vi "Create Numeric Channel.vi"(7 "Input?":bool, 8 "error in (no error)":errorcluster, 10 "Channel Number":i32) -> (0 "error out":errorcluster, 2 "Numeric Channel":T1, 3 "Channel out":refnum<class "Channel.lvclass">)   [LabVIEW 2026, in "Modbus.lvlib" / "Modbus.lvclass"]
uses:
  Modbus.lvclass
  <vilib>/FlexLogger/SDK/PluginSDK.lvlibp/PEFClasses/SDK/Channel/Channel.lvclass
  Types/Numeric Data.ctl
  Types/Modbus Table.ctl
  Types/Numeric Size.ctl
  Types/Numeric Data Type.ctl
  Types/Numeric Location.ctl
  1585c66d-b047-40a8-b383-e25739784f18.vi
  2dd19376-ff6e-472a-aab6-17888e896a0b.vi
  e0cdf0dc-ec87-4ce3-9d59-fa7e6132dbb7.vi
  2dd19376-ff6e-472a-aab6-17888e896a0b.vi/407e0540-03f6-4363-afc5-a4b1f046ef19.vi
  2dd19376-ff6e-472a-aab6-17888e896a0b.vi/520d475a-7b95-4b20-931b-ccc2be82a762.vi
  <vilib>/FlexLogger/SDK/PluginSDK.lvlibp/PEFClasses/SDK/Setpoint Consumer Channel/Setpoint Consumer Channel.lvclass
  <vilib>/FlexLogger/SDK/PluginSDK.lvlibp/PEFClasses/SDK/Producer Channel/Producer Channel.lvclass
  Globals/Modbus Strings.vi
  <vilib>/FlexLogger/SDK/PluginSDK.lvlibp/PEFClasses/SDK/Setpoint Consumer Channel/Create Setpoint Consumer Channel_v2.vi
  <vilib>/FlexLogger/SDK/PluginSDK.lvlibp/PEFClasses/SDK/Producer Channel/Create Producer Channel_v2.vi
  <vilib>/FlexLogger/SDK/PluginSDK.lvlibp/PEFClasses/SDK/Channel/ParameterAccess/Write Enum.vi
  <vilib>/FlexLogger/SDK/PluginSDK.lvlibp/PEFClasses/SDK/Channel/ParameterAccess/Write I32.vi
  <vilib>/FlexLogger/SDK/PluginSDK.lvlibp
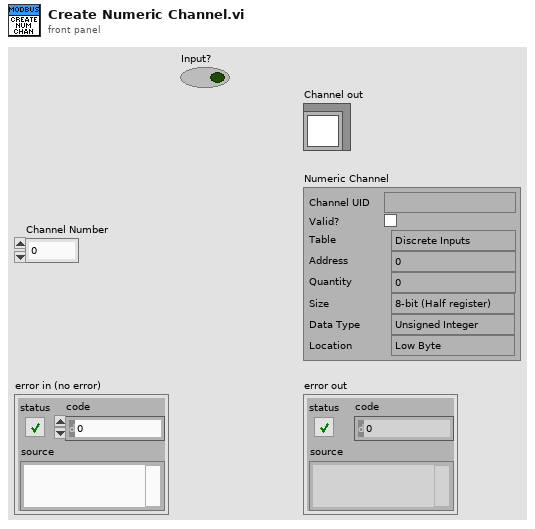
[diagram p1: front panel]
types:
  T1 = typedef "Modbus.lvlib/Modbus.lvclass/Numeric Data.ctl" = cluster{"Channel UID":string, "Valid?":bool, "Table":T2, "Address":i32, "Quantity":u16, "Size":T3, "Data Type":T4, "Location":T5}
  T2 = typedef "Modbus.lvlib/Modbus.lvclass/Modbus Table.ctl" = enum16{"Discrete Inputs", "Coils", "Input Registers", "Holding Registers"}
  T3 = typedef "Modbus.lvlib/Modbus.lvclass/Numeric Size.ctl" = enum16{"8-bit (Half register)", "16-bit (One register)", "32-bit (Two registers)", "64-bit (Four registers)"}
  T4 = typedef "Modbus.lvlib/Modbus.lvclass/Numeric Data Type.ctl" = enum16{"Unsigned Integer", "Signed Integer", "Floating Point"}
  T5 = typedef "Modbus.lvlib/Modbus.lvclass/Numeric Location.ctl" = enum16{"Low Byte", "High Byte"}
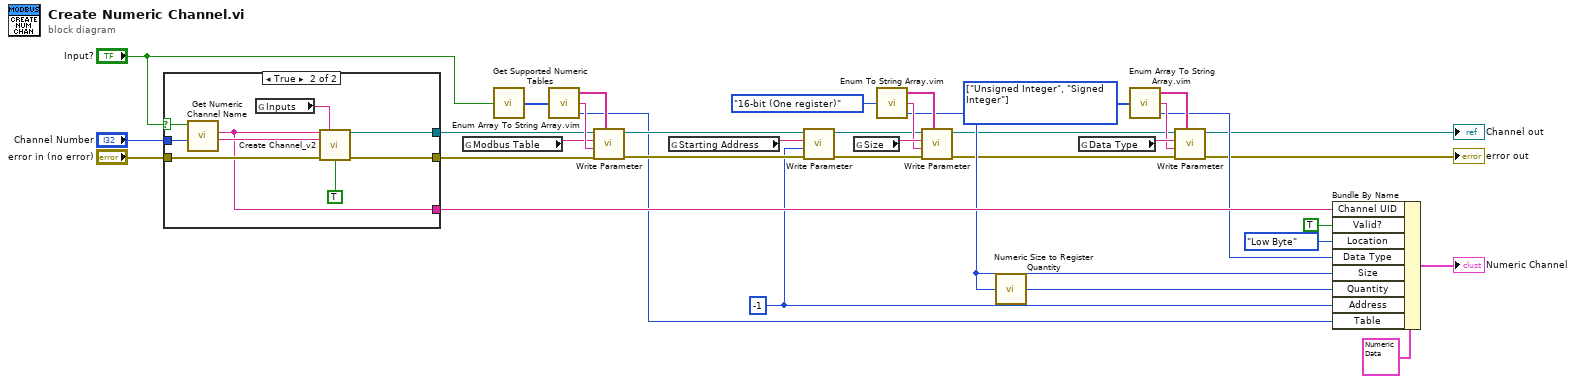
[diagram p0: block diagram]
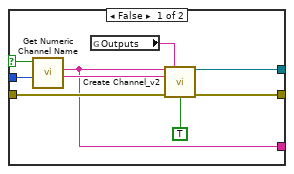
[diagram p2: hidden frame]
diagram:
  w4 = T4[] [enum."Unsigned Integer", enum."Signed Integer"] items=["Unsigned Integer", "Signed Integer", "Floating Point"]
  w20 = -1 ("Value")
  n1 = case shown="True" "Input?" {
    selector: "Input?" -> [w40 w49]
    tunnel: "error in (no error)" -> [w42 w51]
    tunnel: [w44 w53] -> w28
    tunnel: [w45 w54] -> w29
    tunnel: "Channel Number" -> [w37 w46]
    tunnel: [w38 w47] -> w36
    frame False {
      n2 = call "Get Numeric Channel Name.vi"("Channel Numer"=w37, "Input?"=w40) -> ("Num Channel Name"=w39:string, "Num Channel ID"=w38:string)  [unwired: 8 in]
      n3 = global read "Modbus Strings.vi" "Outputs"() -> (w43:string)
      n4 = call-poly <vilib>:"Create Channel_v2.vi"("Unique Channel Identifier"=w38, "Display Group"=w43, "Default Channel Name"=w39, "error in (no error)"=w42, "Can Disable?"=TRUE) -> ("Setpoint Consumer Channel"=w44:refnum<class "Setpoint Consumer Channel.lvclass">, "error out"=w45:errorcluster)  [unwired: 9 in]
    }
    frame True {
      n5 = call "Get Numeric Channel Name.vi"("Channel Numer"=w46, "Input?"=w49) -> ("Num Channel Name"=w48:string, "Num Channel ID"=w47:string)  [unwired: 8 in]
      n6 = global read "Modbus Strings.vi" "Inputs"() -> (w52:string)
      n7 = call-poly <vilib>:"Create Channel_v2.vi"("Unique Channel Identifier"=w47, "Display Group"=w52, "Default Channel Name"=w48, "error in (no error)"=w51, "Can Disable?"=TRUE) -> ("Producer Channel"=w53:refnum<class "Producer Channel.lvclass">, "error out"=w54:errorcluster)  [unwired: 9 in]
    }
  }
  n8 = global read "Modbus Strings.vi" "Modbus Table"() -> (w26:string)
  n9 = call "Get Supported Numeric Tables.vi"("Input?"="Input?") -> ("Supported Tables"=w35:T2[])
  n10 = call "Enum Array To String Array.vim"("Array of Enum Values"=w35) -> ("First Value"=w21:T2, "First String"=w31:string, "Strings out"=w30:string[])  [unwired: 2 in]
  n11 = call-poly <vilib>:"Write Parameter.vi"("Possible Values"=w30, "error in (no error)"=w29, "Current Value"=w31, "Name"=w26, "Channel in"=w28) -> ("error out"=w23:errorcluster, "Channel out"=w22:refnum<class "Channel.lvclass">)  [unwired: 5 in]
  n12 = global read "Modbus Strings.vi" "Starting Address"() -> (w27:string)
  n13 = call-poly <vilib>:"Write Parameter.vi"("error in (no error)"=w23, "Value"=w20, "Name"=w27, "Channel in"=w22) -> ("error out"=w13:errorcluster, "Channel out"=w14:refnum<class "Channel.lvclass">)  [unwired: 6 in]
  n14 = global read "Modbus Strings.vi" "Size"() -> (w17:string)
  n15 = call "Enum To String Array.vim"("Enum in"=Numeric_Size."16-bit (One register)" ("Size")) -> ("Selected Value out"=w10:T3, "Selected String out"=w15:string, "Strings out"=w16:string[])  [unwired: 2 in]
  n16 = call-poly <vilib>:"Write Parameter.vi"("Possible Values"=w16, "error in (no error)"=w13, "Current Value"=w15, "Name"=w17, "Channel in"=w14) -> ("error out"=w5:errorcluster, "Channel out"=w6:refnum<class "Channel.lvclass">)  [unwired: 5 in]
  n17 = call "Numeric Size to Register Quantity.vi"("Size"=w10) -> ("Quantity"=w11:u16)
  n18 = global read "Modbus Strings.vi" "Data Type"() -> (w9:string)
  n19 = call "Enum Array To String Array.vim"("Array of Enum Values"=w4) -> ("First Value"=w3:T4, "First String"=w7:string, "Strings out"=w8:string[])  [unwired: 2 in]
  n20 = call-poly <vilib>:"Write Parameter.vi"("Possible Values"=w8, "error in (no error)"=w5, "Current Value"=w7, "Name"=w9, "Channel in"=w6) -> ("error out"=→"error out":errorcluster, "Channel out"=→"Channel out":refnum<class "Channel.lvclass">)  [unwired: 5 in]
  n21 = Bundle By Name(cluster=T1 {"Channel UID"="", "Valid?"=FALSE, "Table"=enum."Discrete Inputs", "Address"=0, "Quantity"=0, "Size"=enum."8-bit (Half register)", "Data Type"=enum."Unsigned Integer", "Location"=enum."Low Byte"} ("Numeric Data"), "Channel UID"=w36, "Valid?"=TRUE, "Location"=Numeric_Location."Low Byte", "Data Type"=w3, "Size"=w10, "Quantity"=w11, "Address"=w20, "Table"=w21) -> (→"Numeric Channel":T1)
